vi "labview-quick-event.vi"   [LabVIEW 2020]
uses:
  Nominal Client/Nominal Client.lvclass/Nominal Client.ctl
  User/User.lvclass
  Nominal Client/Nominal Client.lvclass
  nominal types/workspace/workspace.lvclass
  submodules/reqwest-labview/lv-src/reqwest/reqwest.lvclass
  e79185ee-863a-4b48-b269-365b27d9e424.vi
  asset/asset.lvclass
  Run/Run.lvclass
  event/event.lvclass
  Nominal Client/asset.get.vi
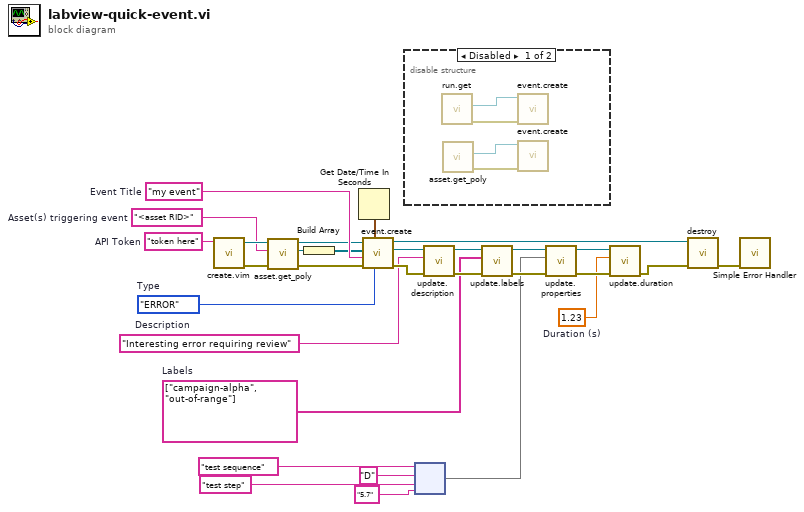
[diagram p0: block diagram]
diagram:
  w1 = "<asset RID>"  # Asset(s) triggering event
  w8 = 1.23  # Duration (s)
  w11 = enum16{"INFO", "FLAG", "ERROR", "SUCCESS"}."ERROR"  # Type
  w19 = string[] ["campaign-alpha", "out-of-range"]  # Labels
  w22 = "Interesting error requiring review"  # Description
  w29 = "token here"  # API Token
  w24 = "my event"  # Event Title
  n1 = call "create.vim"("API Token (string or path)"=w29) -> ("error out"=w7:errorcluster, "Nominal Client"=w6:refnum<class "Nominal Client.lvclass">)  [unwired: 8 in, 1 out]
  n2 = call-poly "asset.get_poly.vi"("error in"=w7, "Asset RID"=w1, "Nominal Client in"=w6) -> ("error out"=w4:errorcluster, "Asset"=w3:refnum<class "asset.lvclass">, "Nominal Client out"=w5:refnum<class "Nominal Client.lvclass">)  [unwired: 6 in]
  n3 = Build Array(w3) -> (w2:refnum<class "asset.lvclass">[])
  n4 = Get Date/Time In Seconds() -> (seconds since 1Jan1904=w10:timestamp)
  n5 = call "event.create.vi"("Type"=w11, "Time Stamp (now: system time)"=w10, "error in"=w4, "Name"=w24, "assets"=w2, "Nominal Client in"=w5) -> ("error out"=w23:errorcluster, "event"=w9:refnum<class "event.lvclass">, "Nominal Client out"=w16:refnum<class "Nominal Client.lvclass">)  [unwired: 3 in]
  n6 = disable-structure shown="Disabled" {
    frame Disabled {
      n7 = call "run.get.vi"() -> ("error out"=w31:errorcluster, "Run"=w32:refnum<class "Run.lvclass">)  [unwired: 9 in, 1 out]
      n8 = call-poly "asset.get_poly.vi"() -> ("error out"=w34:errorcluster, "Asset"=w33:refnum<class "asset.lvclass">)  [unwired: 9 in, 1 out]
      n9 = call "event.create.vi"("error in (no error)"=w31, "Run in"=w32) -> ()  [unwired: 7 in, 3 out]
      n10 = call "event.create.vi"("error in"=w34, "asset in"=w33) -> ()  [unwired: 7 in, 3 out]
    }
    frame Enabled {
    }
  }
  n11 = node("test sequence", "D", "test step", "5.7") -> (w15:map{string, string})
  n12 = call "update.description.vi"("error in (no error)"=w23, "Name"=w22, "event in"=w9) -> ("error out"=w20:errorcluster, "event out"=w21:refnum<class "event.lvclass">)  [unwired: 7 in]
  n13 = call "update.labels.vi"("error in (no error)"=w20, "Labels"=w19, "event in"=w21) -> ("error out"=w17:errorcluster, "event out"=w18:refnum<class "event.lvclass">)  [unwired: 7 in]
  n14 = call "update.properties.vi"("error in (no error)"=w17, "properties"=w15, "event in"=w18) -> ("error out"=w14:errorcluster, "event out"=w13:refnum<class "event.lvclass">)  [unwired: 7 in]
  n15 = call "update.duration.vi"("error in (no error)"=w14, "Duration (s)"=w8, "event in"=w13) -> ("error out"=w12:errorcluster)  [unwired: 7 in, 1 out]
  n16 = call "destroy.vi"("error in"=w12, "Nominal Client"=w16) -> ("error out"=w30:errorcluster)  [unwired: 9 in]
  n17 = call <vilib>:"Simple Error Handler.vi"("error in (no error)"=w30) -> ()  [unwired: 4 in, 5 out]
